vi "New Lua State.vi"(6 "open libs? (T)":bool=TRUE, 8 "error in (no error)":errorcluster) -> (0 "error out":errorcluster, 3 "Lua out":refnum<class "Lua.lvclass">)   [LabVIEW 2020, in "Lua for LabVIEW.lvlib" / "Lua.lvclass"]
doc: "Creates a new Lua state. \n\nDefaults to open all standard Lua libraries."
uses:
  Lua.lvclass
  private/lua_monitor_event.ctl
  Lua.lvclass/Lua.ctl
  private/lua_monitor.vi
  lib/lua.dll/lua.dll.lvlib
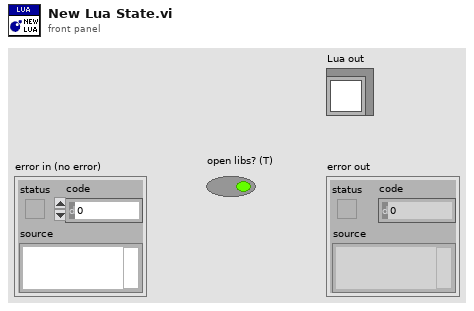
[diagram p1: front panel]
types:
  T1 = typedef "Lua for LabVIEW.lvlib/Lua.lvclass/lua_monitor_event.ctl" = enum16{"<null>", "terminate"}
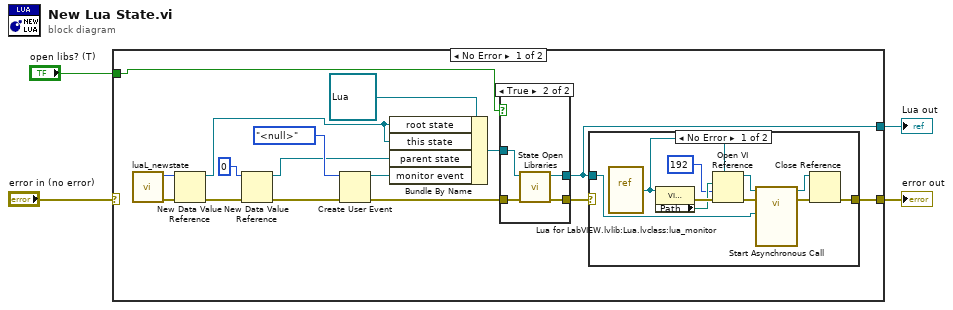
[diagram p0: block diagram]
diagram:
  n1 = case shown="No Error" "error in (no error)" {
    selector: "error in (no error)" -> [_ w38]
    tunnel: [w17 w38] -> w3
    tunnel: "open libs? (T)" -> [w15 _]
    tunnel: [w5 _] -> w1
    frame No Error {
      n2 = call "luaL_newstate.vi"() -> ("error out"=w11:errorcluster, "lua_state_p"=w10:u64)  [unwired: 10 in]
      n3 = New Data Value Reference(data value=w10, error in=w11) -> (data value reference=w9:refnum<data-value>, error out=w7:errorcluster)
      n4 = New Data Value Reference(data value=u64 0, error in=w7) -> (data value reference=w8:refnum<data-value>, error out=w13:errorcluster)
      n5 = Create User Event(user event datatype=lua_monitor_event."<null>" ("event"), error in=w13) -> (user event=w18:refnum<user-event>, error out=w12:errorcluster)
      n6 = Bundle By Name(cluster=refnum<class "Lua.lvclass"> refnum ("Lua in"), "root state"=w9, "this state"=w9, "parent state"=w8, "monitor event"=w18) -> (w16:refnum<class "Lua.lvclass">)
      n7 = case shown="True" w15 {
        tunnel: w16 -> [w22 w26]
        tunnel: [w22 w25] -> w5
        tunnel: [w21 w24] -> w6
        tunnel: w12 -> [w21 w23]
        frame False {
        }
        frame True {
          n8 = call-dynamic "State Open Libraries.vi"("error in (no error)"=w23, "Lua in"=w26) -> ("error out"=w24:errorcluster, "Lua out"=w25:refnum<class "Lua.lvclass">)  [unwired: 8 in]
        }
      }
      n9 = case shown="No Error" w6 {
        selector: w6 -> [_ w37]
        tunnel: [w28 w37] -> w17
        tunnel: w5 -> [w27 _]
        frame No Error {
          n10 = vi-ref "Lua for LabVIEW.lvlib:Lua.lvclass:lua_monitor.vi"() -> (w35:refnum<vi>)
          n11 = property class="VI (strict)"(reference=w35) -> (error out=w36:errorcluster, "Path"=w34:path)  [unwired: 1 in, 1 out]
          n12 = Open VI Reference(type specifier VI Refnum (for type only)=w35, vi path=w34, options=192, error in (no error)=w36) -> (vi reference=w32:refnum<vi>, error out=w31:errorcluster)  [unwired: 2 in]
          n13 = call-by-ref "Start Asynchronous Call"(reference=w32, error in=w31, "Lua for LabVIEW.lvlib:Lua.lvclass"=w27) -> (reference out=w30:refnum<vi>, error out=w29:errorcluster)  [unwired: 11 in]
          n14 = Close Reference(reference=w30, error in (no error)=w29) -> (error out=w28:errorcluster)
        }
        frame Error {
        }
      }
    }
    frame Error {
    }
  }
  "error out" <- w3
  "Lua out" <- w1
